vi "PicoScope6000Open.vi"(3 "Serial Number":string, 4 "error in (no error)":errorcluster, 5 "Use Serial Number":bool) -> (0 "handle":i16, 1 "Max Adc value":i16, 2 "error out":errorcluster, 6 "Device Info":T1)   [LabVIEW 2016]
doc: "This VI opens a PicoScope 6000 and returns a handle to the device."
uses:
  ps6000.dll
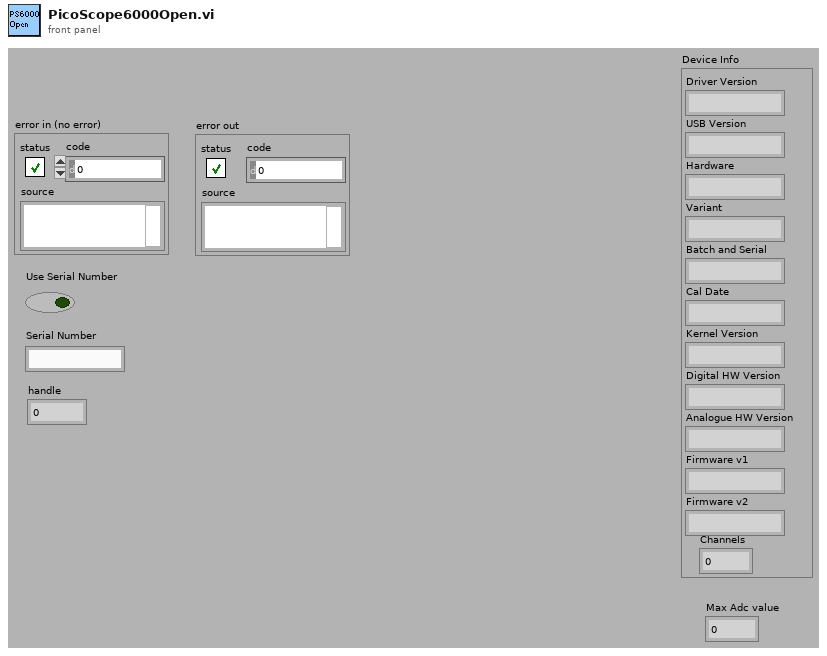
[diagram p1: front panel]
types:
  T1 = cluster{"Driver Version":string, "USB Version":string, "Hardware":string, "Variant":string, "Batch and Serial":string, "Cal Date":string, "Kernel Version":string, "Digital HW Version":string, "Analogue HW Version":string, "Firmware v1":string, "Firmware v2":string, "Channels":i16}
  T2 = cluster{"Driver Version":string, "USB Version":string, "Hardware":string, "Variant":string, "Batch and Serial":string, "Cal Date":string, "Kernel Version":string, "Digital HW Version":string, "Analogue HW Version":string, "Firmware v1":string, "Firmware v2":string}
  T3 = cluster{"Driver Version":string, "USB Version":string, "Hardware":string, "Variant":string, "Batch and Serial":string, "Cal Date":string, "Kernel Version":string, "Digital HW Version":string, "Analogue HW Version":string, "Firmware v1":string, "Firmware v2":string, i16}
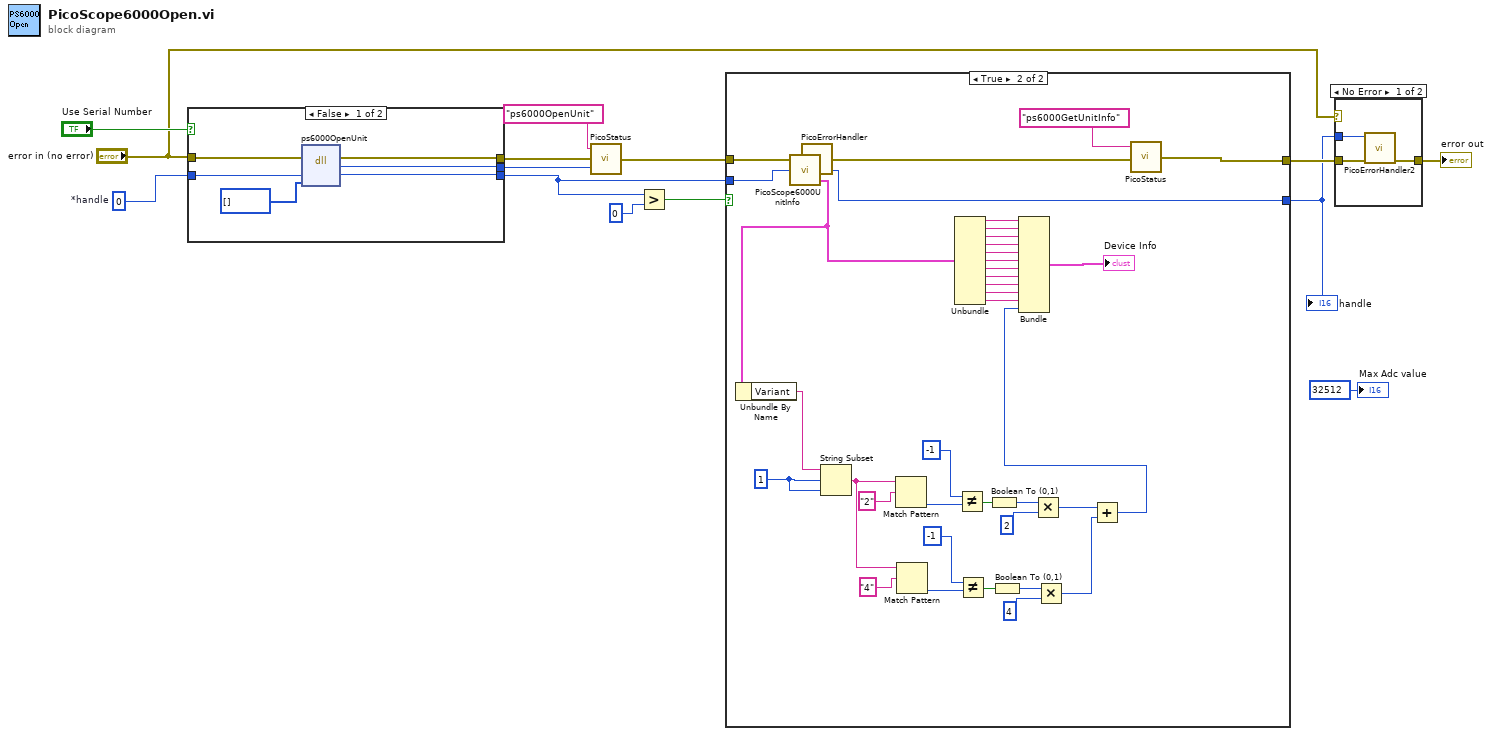
[diagram p0: block diagram]
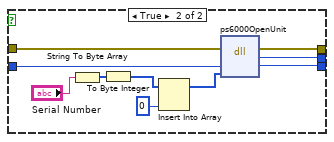
[diagram p4: hidden frame]
diagram:
  w12 = i16 0  # *handle
  n1 = case shown="False" "Use Serial Number" {
    tunnel: "error in (no error)" -> [w20 w26]
    tunnel: w12 -> [w19 w27]
    tunnel: [w18 w30] -> w11
    tunnel: [w17 w29] -> w10
    tunnel: [w16 w28] -> w6
    frame False {
      n2 = dll-call lib="PS6000.dll" fn="ps6000OpenUnit" ("ps3000.dll:_ps3000_open_unit@0")(error in=w20, "handle"=w19, "serial"=i8[] []) -> (error out=w18:errorcluster, "PICO_STATUS"=w17:u32, "handle"=w16:i16)  [unwired: 3 in, 1 out]
    }
    frame True {
      n3 = String To Byte Array(string="Serial Number") -> (unsigned byte array=w24:u8[])
      n4 = To Byte Integer(number=w24) -> (8bit integer=w25:i8[])
      n5 = Insert Into Array(array=w25, new element=i8 0 ("new element/subarray")) -> (w21:i8[])  [unwired: 1 in]
      n6 = dll-call lib="PS6000.dll" fn="ps6000OpenUnit" ("ps3000.dll:_ps3000_open_unit@0")(error in=w26, "handle"=w27, "serial"=w21) -> (error out=w30:errorcluster, "PICO_STATUS"=w29:u32, "handle"=w28:i16)  [unwired: 3 in, 1 out]
    }
  }
  n7 = call "PicoStatus.vi"("PICO STATUS"=w10, "error in"=w11, "source"="ps6000OpenUnit") -> ("error out"=w8:errorcluster)
  n8 = Greater?(x=w6, y=0) -> (0:w7:bool)
  n9 = case shown="True" w7 {
    tunnel: w6 -> [w31 w69]
    tunnel: w8 -> [w32 w68]
    tunnel: [w32 w66] -> w5
    tunnel: [w31 w64] -> w1
    frame False {
    }
    frame True {
      w51 = 1 ("offset (0)")
      n10 = call "PicoScope6000UnitInfo.vi"("handle in"=w69, "error in (no error)"=w68) -> ("Unit Info"=w63:T2, "handle out"=w64:i16, "error out"=w67:errorcluster)  [unwired: 1 in]
      n11 = Unbundle By Name(w63) -> ("Variant"=w35:string)
      n12 = String Subset(string=w35, offset (0)=w51, length (rest)=w51) -> (substring=w44:string)
      n13 = Match Pattern(string=w44, regular expression="2") -> (offset past match=w49:i32)  [unwired: 1 in, 3 out]
      n14 = Match Pattern(string=w44, regular expression="4") -> (offset past match=w46:i32)  [unwired: 1 in, 3 out]
      n15 = Unbundle(w63) -> ("Driver Version"=w62:string, "USB Version"=w61:string, "Hardware"=w60:string, "Variant"=w59:string, "Batch and Serial"=w58:string, "Cal Date"=w57:string, "Kernel Version"=w56:string, "Digital HW Version"=w55:string, "Analogue HW Version"=w54:string, "Firmware v1"=w53:string, "Firmware v2"=w52:string)
      n16 = Not Equal?(x=-1, y=w49) -> (x != y?=w41:bool)
      n17 = Not Equal?(x=-1, y=w46) -> (x != y?=w37:bool)
      n18 = Boolean To (0,1)(Boolean=w41) -> (0, 1=w40:i16)
      n19 = Boolean To (0,1)(Boolean=w37) -> (0, 1=w38:i16)
      n20 = Multiply(x=w40, y=i16 2) -> (x*y=w43:i16)
      n21 = Multiply(x=w38, y=i16 4) -> (x*y=w36:i16)
      n22 = Add(x=w43, y=w36) -> (x+y=w34:i16)
      n23 = Bundle("Driver Version"=w62, "USB Version"=w61, "Hardware"=w60, "Variant"=w59, "Batch and Serial"=w58, "Cal Date"=w57, "Kernel Version"=w56, "Digital HW Version"=w55, "Analogue HW Version"=w54, "Firmware v1"=w53, "Firmware v2"=w52, w34) -> (→"Device Info":T3)  [unwired: 1 in]
      n24 = call "PicoStatus.vi"("error in"=w67, "source"="ps6000GetUnitInfo") -> ("error out"=w66:errorcluster)  [unwired: 1 in]
    }
  }
  "handle" <- w1
  n25 = call "PicoErrorHandler.vi"() -> ()  [unwired: 1 in, 1 out]
  n26 = case shown="No Error" "error in (no error)" {
    tunnel: [w72 w73] -> w4
    tunnel: w5 -> [w71 w73]
    tunnel: w1 -> [w70 _]
    frame No Error {
      n27 = call "PicoErrorHandler2.vi"("error in (no error)"=w71, "handle In"=w70) -> ("error out"=w72:errorcluster)  [unwired: 9 in]
    }
    frame Error {
    }
  }
  "error out" <- w4
  "Max Adc value" <- i16 32512 ("Max Adc value")
